vi "Inspector Launcher [VarMan Spy].vi"(5 "VC Handle":T1=-1, 9 "Variable":string) -> (0 "error out":errorcluster)   [LabVIEW 2021]
doc: "::: CalcExpress Toolkit :::\nCopyright (c) 2000-2026 Konstantin Shifershteyn. All rights reserved."
uses:
  vi.lib/addons/CalcExpress/cetypes.llb/VarMan Variable Context Handle.ctl
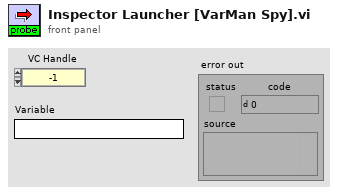
[diagram p1: front panel]
types:
  T1 = typedef "VarMan Variable Context Handle.ctl" = i32
  T2 = enum32{"Invalid", "Standard", "Closed", "Hidden", "Minimized", "Maximized"}
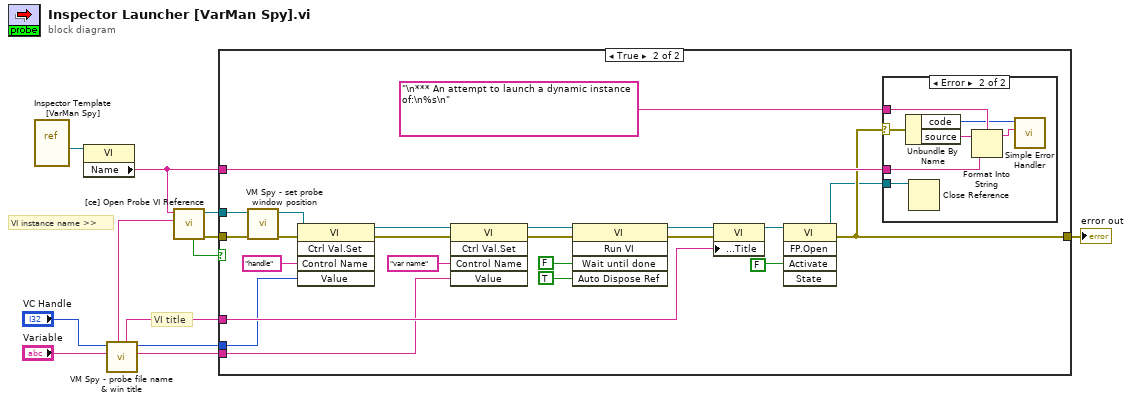
[diagram p0: block diagram]
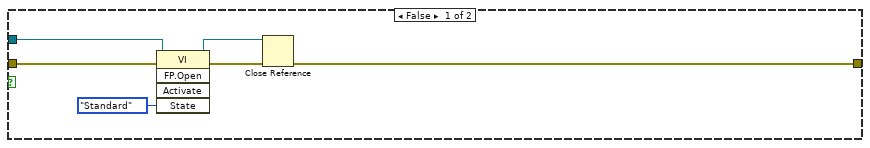
[diagram p2: hidden frame]
diagram:
  # "VI title"
  # "VI instance name >>"
  n1 = vi-ref "Inspector Template [VarMan Spy].vi"() -> (w1:refnum<vi>)
  n2 = property class="VI"(reference=w1) -> ("Name"=w2:string)  [unwired: 1 in, 2 out]
  n3 = call "VM Spy - probe file name & win title.vi"("Variable"="Variable", "VC Handle"="VC Handle") -> ("var name"=w9:string, "VC Handle out"=w10:T1, "probe win title"=w11:string, "probe instance name"=w4:string)  [unwired: 3 in, 1 out]
  n4 = call "[ce] Open Probe VI Reference.vi"("VI instance name"=w4, "master VI name"=w2) -> ("error out"=w3:errorcluster, "vi refnum"=w6:refnum<vi>, "new window?"=w5:bool)  [unwired: 7 in]
  n5 = case shown="True" w5 {
    tunnel: w10 -> [_ w25]
    tunnel: w9 -> [_ w24]
    tunnel: [w16 w21] -> w12
    tunnel: w6 -> [w15 w29]
    tunnel: w11 -> [_ w30]
    tunnel: w3 -> [w14 w28]
    tunnel: w2 -> [_ w27]
    frame False {
      n6 = invoke class="VI" method="FP.Open"(reference=w15, error in=w14, "State"=T2."Standard") -> (reference out=w17:refnum<vi>, error out=w18:errorcluster)  [unwired: 2 in, 3 out]
      n7 = Close Reference(reference=w17, error in (no error)=w18) -> (error out=w16:errorcluster)
    }
    frame True {
      n8 = call "VM Spy - set probe window position.vi"("error in"=w28, "refnum"=w29) -> ("error out"=w34:errorcluster, "dup refnum"=w33:refnum<vi>)  [unwired: 6 in]
      n9 = invoke class="VI" method="Ctrl Val.Set"(reference=w33, error in=w34, "Control Name"="handle", "Value"=w25) -> (reference out=w38:refnum<vi>, error out=w39:errorcluster)  [unwired: 1 in, 3 out]
      n10 = invoke class="VI" method="Ctrl Val.Set"(reference=w38, error in=w39, "Control Name"="var name", "Value"=w24) -> (reference out=w31:refnum<vi>, error out=w32:errorcluster)  [unwired: 1 in, 3 out]
      n11 = invoke class="VI" method="Run VI"(reference=w31, error in=w32, "Wait until done"=FALSE, "Auto Dispose Ref"=TRUE ("Auto Dispose Reference")) -> (reference out=w35:refnum<vi>, error out=w36:errorcluster)  [unwired: 1 in, 3 out]
      n12 = property class="VI"(reference=w35, error in=w36, "Front Panel Window:Title"=w30) -> (reference out=w22:refnum<vi>)  [unwired: 1 out]
      n13 = invoke class="VI" method="FP.Open"(reference=w22, "Activate"=FALSE) -> (reference out=w20:refnum<vi>, error out=w21:errorcluster)  [unwired: 3 in, 3 out]
      n14 = case shown="Error" w21 {
        selector: w21 -> [_ w43]
        tunnel: w27 -> [_ w47]
        tunnel: "\n*** An attempt to launch a dynamic instance of:\n%s\n" -> [_ w46]
        tunnel: w20 -> [_ w42]
        frame No Error {
        }
        frame Error {
          n15 = Unbundle By Name(w43) -> ("code"=w45:i32, "source"=w48:string)
          n16 = Close Reference(reference=w42) -> ()  [unwired: 1 in, 1 out]
          n17 = Format Into String(format string=w46, initial string=w48, w47) -> (resulting string=w44:string)  [unwired: 1 in, 1 out]
          n18 = call <vilib>:"Simple Error Handler.vi"("error code (no error:0)"=w45, "error source (\" \")"=w44) -> ()  [unwired: 3 in, 5 out]
        }
      }
    }
  }
  "error out" <- w12
